vi "Create Redirect Response.vi"   [LabVIEW 2020]
uses:
  lv-http-util/HTTP Utils/Redirect Response/Redirect Response.lvclass
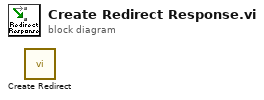
[diagram p0: block diagram]
diagram:
  n1 = call "Create Redirect.vi"() -> ()  [unwired: 10 in, 2 out]
